vi "GEvt-Generate Complete Log.vi"(0 "CSM Global Log Event":T4, 2 "Event Data":T1={"Name (\"\" to Use UUID)"="", "Current State"="", "Arguments"="", "Source Message"={"‘State"="", "’Arguments"="", "’Error"={"status"=FALSE, "code"=0, "source"=""}}, "Source Module"="", "Complete(T)/Start(F)"=FALSE, "LogType"=enum."State Change", "Time Stamp"=timestamp(0 s since 1904-01-01)}, 7 "Enable?":bool=TRUE, 10 "CSM:LogFilter.lvclass":refnum<class "LogFilter.lvclass">) -> (14 "CSM Global Log Event Out":T4)   [LabVIEW 2017, in "Communicable State Machine.lvlib"]
doc: "### GEvt-Generate Complete Log.vi\n\n-- <b>Controls</b> --\n- <b>CSM Global Log Event</b>:\n- <b>event data</b>:\n- <b>Enable?</b>:\n- <b>CSM:LogFilter.lvclass</b>:\n\n-- <b>Indicators</b> --\n- <b>CSM Global Log Event out</b>:"
uses:
  Communicable State Machine.lvlib
  GEvt-Refs.ctl
  Typedef/_CSM_GlobalLog_MSG.ctl
  Typedef/_CSM_Response Source Message.ctl
  Typedef/_CSM_GlobalLog_MSG_TYPE.ctl
  LogFilter/LogFilter.lvclass
  LogFilter/LogFilter - Check.vi
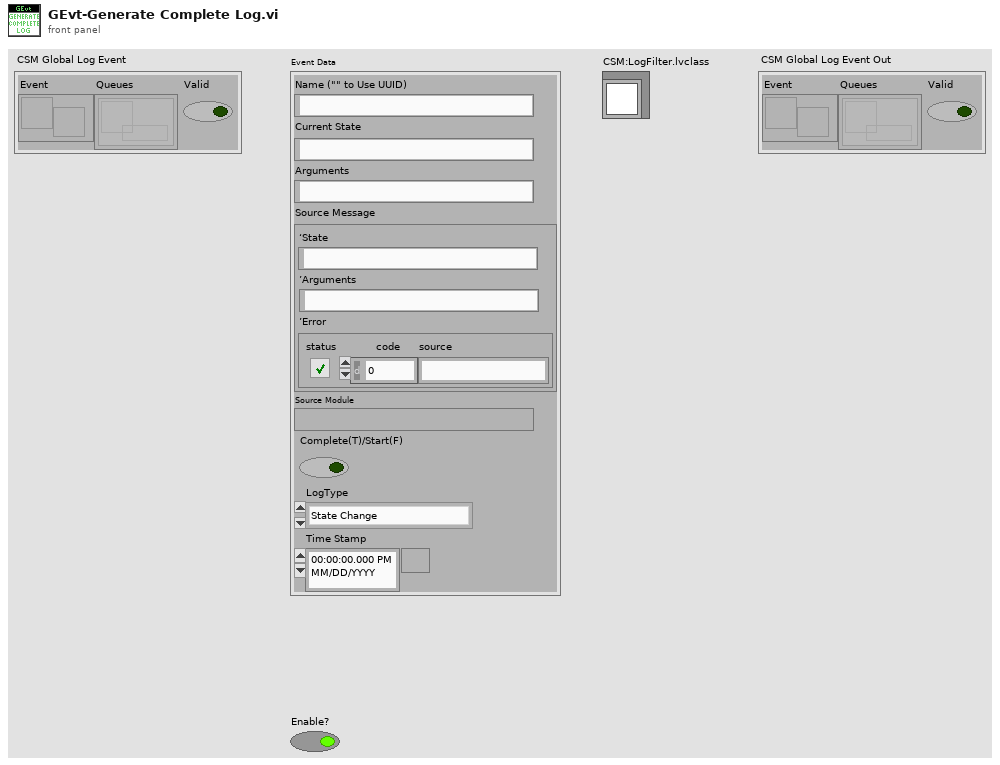
[diagram p1: front panel]
types:
  T1 = typedef "Communicable State Machine.lvlib/_CSM_GlobalLog_MSG.ctl" = cluster{"Name (\"\" to Use UUID)":string, "Current State":string, "Arguments":string, "Source Message":T2, "Source Module":string, "Complete(T)/Start(F)":bool, "LogType":T3, "Time Stamp":timestamp}
  T2 = typedef "Communicable State Machine.lvlib/_CSM_Response Source Message.ctl" = cluster{"‘State":string, "’Arguments":string, "’Error":errorcluster}
  T3 = typedef "Communicable State Machine.lvlib/_CSM_GlobalLog_MSG_TYPE.ctl" = enum16{"User Log", "State Change", "Status", "Interrupt", "Register", "Unregister", "Error Log", "Module Created", "Module Destroyed", "Async Message", "No-Rep Async Message", "Sync Message"}
  T4 = typedef "Communicable State Machine.lvlib/GEvt-Refs.ctl" = cluster{"Event":refnum<user-event>, "Queues":refnum<queue>[], "Valid":bool}
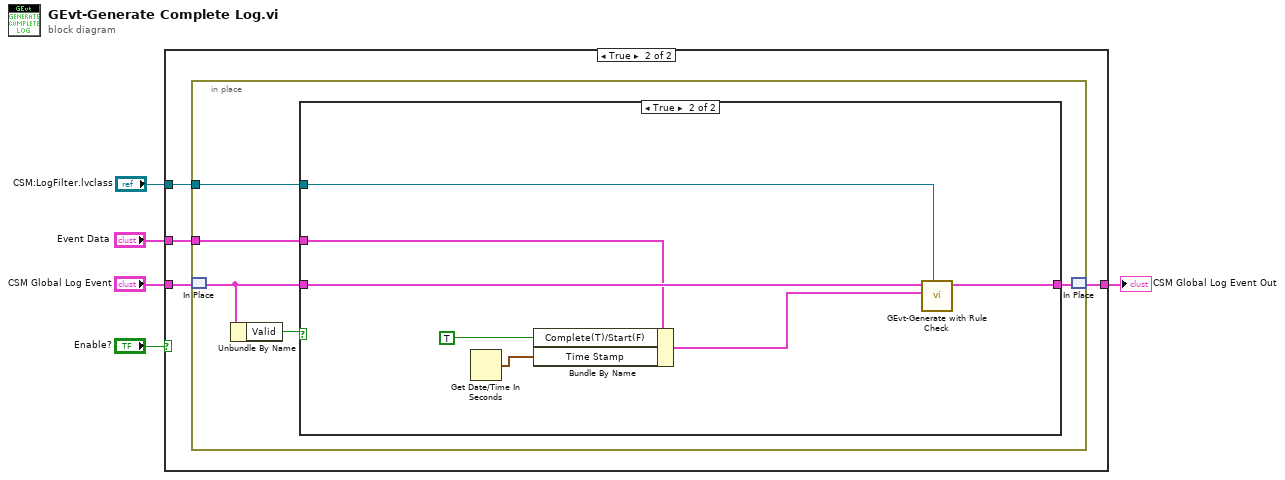
[diagram p0: block diagram]
diagram:
  n1 = case shown="True" "Enable?" {
    tunnel: "CSM Global Log Event" -> [w6 w10]
    tunnel: [w6 w9] -> w4
    tunnel: "Event Data" -> [_ w8]
    tunnel: "CSM:LogFilter.lvclass" -> [_ w7]
    frame False {
    }
    frame True {
      n2 = in-place {
        in-place-border: w8 -> [w14]
        in-place-border: w7 -> [w13]
        n3 = in-place-match #1(w10) -> (w12:T4)
        n4 = Unbundle By Name(w12) -> ("Valid"=w11:bool)
        n5 = case shown="True" w11 {
          tunnel: w12 -> [w16 w23]
          tunnel: [w16 w22] -> w15
          tunnel: w14 -> [_ w21]
          tunnel: w13 -> [_ w20]
          frame False {
          }
          frame True {
            n6 = Get Date/Time In Seconds() -> (seconds since 1Jan1904=w17:timestamp)
            n7 = Bundle By Name(cluster=w21, "Complete(T)/Start(F)"=TRUE, "Time Stamp"=w17) -> (w18:T1)
            n8 = call "GEvt-Generate with Rule Check.vi"("LogFilter In"=w20, "Event Data"=w18, "CSM Global Log Event In"=w23) -> ("CSM Global Log Event Out"=w22:T4)  [unwired: 8 in]
          }
        }
        n9 = in-place-match #1(w15) -> (w9:T4)
      }
    }
  }
  "CSM Global Log Event Out" <- w4
